vi "Posicions aleatories Temps extra.vi"() -> (2 "x":dbl, 3 "y":dbl)   [LabVIEW 2023]
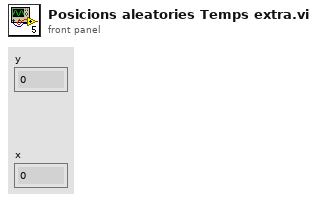
[diagram p1: front panel]
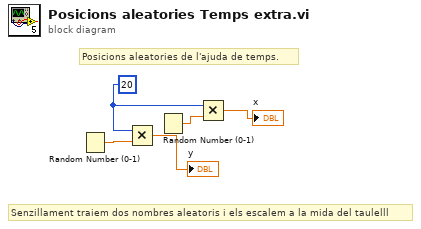
[diagram p0: block diagram]
diagram:
  w5 = 20
  # "Senzillament traiem dos nombres aleatoris i els escalem a la mida del taulelll"
  # "Posicions aleatories de l'ajuda de temps."
  n1 = Random Number (0-1)() -> (number: 0 to 1=w1:dbl)
  n2 = Multiply(x=w5, y=w1) -> (x*y=→"y":dbl)
  n3 = Random Number (0-1)() -> (number: 0 to 1=w2:dbl)
  n4 = Multiply(x=w5, y=w2) -> (x*y=→"x":dbl)
